vi "Execute.vi"(8 "error in (no error)":errorcluster, 9 "Consumer Queues in":T1, 10 "DAC Process Command in":refnum<class "Exit DAC.lvclass">, 11 "DAC Process Data in":T2) -> (0 "error out":errorcluster, 1 "Consumer Queues out":T1, 2 "Stop?":bool, 3 "DAC Process Data out":T2)   [LabVIEW 2019, in "DAC Process.lvlib" / "Exit DAC.lvclass"]
uses:
  Exit DAC.lvclass
  DAC Process Data.ctl
  Generic Test Stand/Generic Test Stand.lvclass
  TS Framework/ExeLogging/DAC Logger/DAC Logger.lvclass
  DAC State.ctl
  TS Framework/Consumer Queues.ctl
  UI Process/Generic UI Command/Generic UI Process Command.lvclass
  Generic DAC Command/Generic DAC Process Command.lvclass
  Trig Process/Generic Trig Command/Generic Trig Process Command.lvclass
  UI Process/Stop UI Process/Stop UI Process.lvclass
  Trig Process/Exit TRIG/Exit TRIG.lvclass
  Generic Test Stand/Generic Test Stand.lvclass/Generic Test Stand.ctl
  DAC Process.lvlib
  TS Framework/TS Framework.lvlib
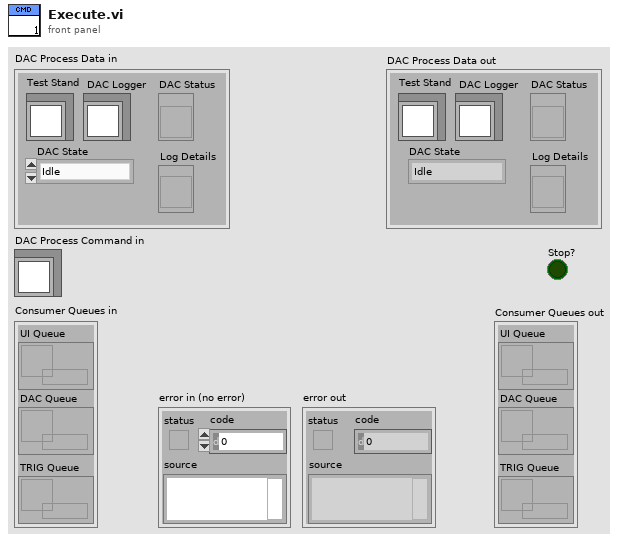
[diagram p1: front panel]
types:
  T1 = typedef "TS Framework.lvlib/Consumer Queues.ctl" = cluster{"UI Queue":refnum<queue>, "DAC Queue":refnum<queue>, "TRIG Queue":refnum<queue>}
  T2 = typedef "DAC Process.lvlib/DAC Process Data.ctl" = cluster{"Test Stand":refnum<class "Generic Test Stand.lvclass">, " DAC Logger":refnum<class "DAC Logger.lvclass">, "DAC State":T3, "DAC Status":refnum<vi>, "Log Details":refnum<vi>}
  T3 = typedef "DAC Process.lvlib/DAC State.ctl" = enum16{"Idle", "Acquiring"}
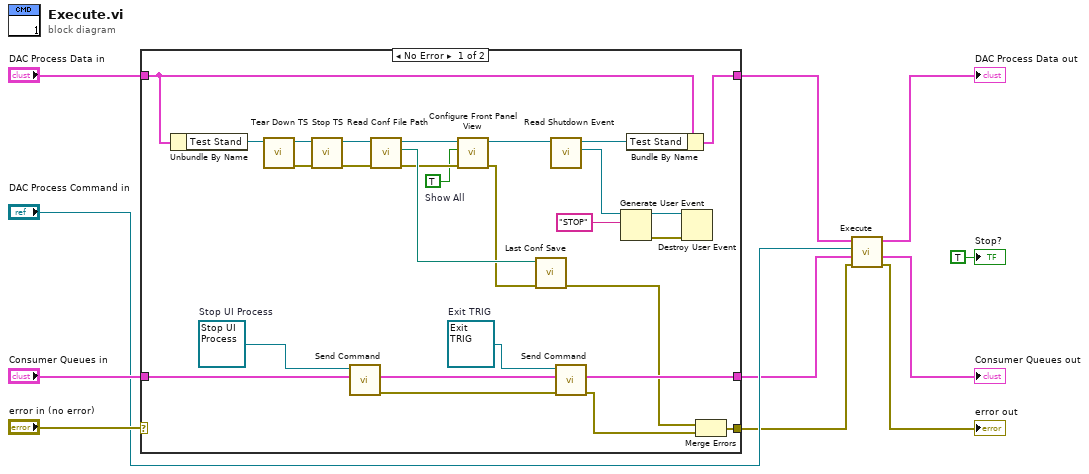
[diagram p0: block diagram]
diagram:
  n1 = case shown="No Error" "error in (no error)" {
    selector: "error in (no error)" -> [_ w41]
    tunnel: [w31 w41] -> w5
    tunnel: "DAC Process Data in" -> [w25 w40]
    tunnel: [w23 w40] -> w4
    tunnel: "Consumer Queues in" -> [w38 w39]
    tunnel: [w35 w39] -> w6
    frame No Error {
      w12 = TRUE  # Show All
      w27 = refnum<class "Exit TRIG.lvclass"> refnum  # Exit TRIG
      w37 = refnum<class "Stop UI Process.lvclass"> refnum  # Stop UI Process
      n2 = Unbundle By Name(w25) -> ("Test Stand"=w26:refnum<class "Generic Test Stand.lvclass">)
      n3 = call-dynamic "Tear Down TS.vi"("Generic Test Stand in"=w26) -> ("error out"=w20:errorcluster, "Generic Test Stand out"=w22:refnum<class "Generic Test Stand.lvclass">)  [unwired: 9 in]
      n4 = call-dynamic "Stop TS.vi"("error in (no error)"=w20, "Generic Test Stand in"=w22) -> ("error out"=w15:errorcluster, "Generic Test Stand out"=w21:refnum<class "Generic Test Stand.lvclass">)  [unwired: 8 in]
      n5 = call-dynamic "Send Command.vi"("Consumer Queues in"=w38, "UI Process Command in"=w37) -> ("error out"=w29:errorcluster, "Consumer Queues out"=w36:T1)  [unwired: 8 in]
      n6 = call "Read Conf File Path.vi"("error in"=w15, "Generic Test Stand in"=w21) -> ("error out"=w14:errorcluster, "Conf File Path"=w28:path, "Generic Test Stand out"=w17:refnum<class "Generic Test Stand.lvclass">)  [unwired: 7 in]
      n7 = call-dynamic "Configure Front Panel View.vi"("error in"=w14, "Show All"=w12, "Generic Test Stand in"=w17) -> ("error out"=w13:errorcluster, "Generic Test Stand out"=w16:refnum<class "Generic Test Stand.lvclass">)  [unwired: 7 in]
      n8 = call "Last Conf Save.vi"("error in"=w13, "Conf File"=w28) -> ("error out"=w19:errorcluster)  [unwired: 8 in]
      n9 = call "Read Shutdown Event.vi"("Generic Test Stand in"=w16) -> ("Shutdown Event"=w34:refnum<user-event>, "Generic Test Stand out"=w24:refnum<class "Generic Test Stand.lvclass">)  [unwired: 8 in, 1 out]
      n10 = call-dynamic "Send Command.vi"("error in (no error)"=w29, "Consumer Queues in"=w36, "Trig Process Command"=w27) -> ("error out"=w30:errorcluster, "Consumer Queues out"=w35:T1)  [unwired: 7 in]
      n11 = Generate User Event(user event=w34, event data cluster="STOP" ("event data")) -> (user event out=w32:refnum<user-event>, error out=w18:errorcluster)  [unwired: 2 in]
      n12 = Bundle By Name(cluster=w25, "Test Stand"=w24) -> (w23:T2)
      n13 = Destroy User Event(user event=w32, error in=w18) -> ()  [unwired: 1 out]
      n14 = Merge Errors(w19, w30) -> (w31:errorcluster)
    }
    frame Error {
    }
  }
  n15 = call-parent "Execute.vi"("error in"=w5, "Consumer Queues in"=w6, "DAC Process Command in"="DAC Process Command in", "DAC Process Data in"=w4) -> ("error out"=→"error out":errorcluster, "Consumer Queues out"=→"Consumer Queues out":T1, "DAC Process Data out"=→"DAC Process Data out":T2)  [unwired: 4 in, 1 out]
  "Stop?" <- TRUE ("Stop?")
